vi "VIH Utility - FILE - Get Path Attributes (Empty-NAP-Rel).vi"(11 "Path":path) -> (0 "Not A Path or Empty path":bool, 1 "Relative path":bool, 3 "dup Path":path, 4 "Not A Path":bool, 5 "Empty path":bool)   [LabVIEW 2014]
doc: "::: VI Helpeks :::\nCopyright (c) 2000-2026 Konstantin Shifershteyn. All rights reserved."
panel:
  # "VI Helpeks\nCopyright (c) 2012-2026 Konstantin Shifershteyn"
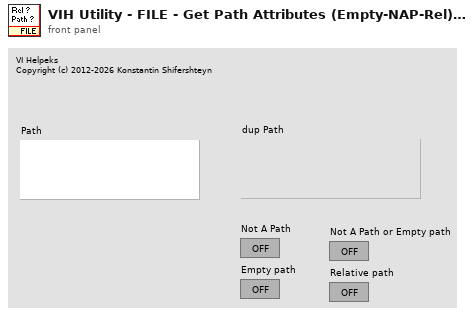
[diagram p1: front panel]
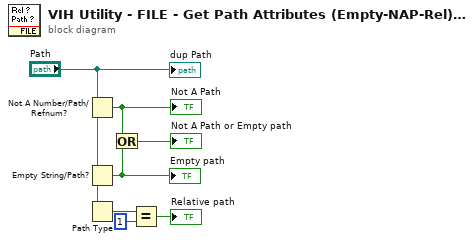
[diagram p0: block diagram]
diagram:
  n1 = Not A Number/Path/Refnum?(number/path/refnum="Path") -> (NaN/Path/Refnum?=w1:bool)
  "Not A Path" <- w1
  n2 = Empty String/Path?(string/path="Path") -> (empty?=w2:bool)
  "Empty path" <- w2
  n3 = Path Type(1:"Path") -> (0:w5:i16)
  n4 = Or(x=w1, y=w2) -> (x .or. y?=→"Not A Path or Empty path":bool)
  n5 = Equal?(x=w5, y=i16 1) -> (x = y?=→"Relative path":bool)
  "dup Path" <- "Path"
